vi "Event Handler.vi"(8 "error in":errorcluster, 11 "Listbox in":refnum<class "Multi Column Listbox.lvclass">) -> (0 "error out":errorcluster, 3 "Listbox out":refnum<class "Multi Column Listbox.lvclass">)   [LabVIEW 2013, in "Table Manager.lvlib" / "Multi Column Listbox.lvclass"]
doc: "Contains a loop and event structure to handle all common MCLB user interactions."
uses:
  Multi Column Listbox.lvclass
  Multi Column Listbox.lvclass/Multi Column Listbox.ctl
  Table Manager/Table Manager.lvclass/Table Manager.ctl
  <vilib>/Utility/miscctls.llb/LVPositionTypeDef.ctl
  <vilib>/Utility/miscctls.llb/LVRowAndColumnTypeDef.ctl
  Table Manager/Menu Select.ctl
  Table Manager/Read object refs.vi
  Table Manager/Read Menu Selection.vi
  Table Manager.lvlib
  Table Manager/Table Manager.lvclass
panel:
  out "Char":i16
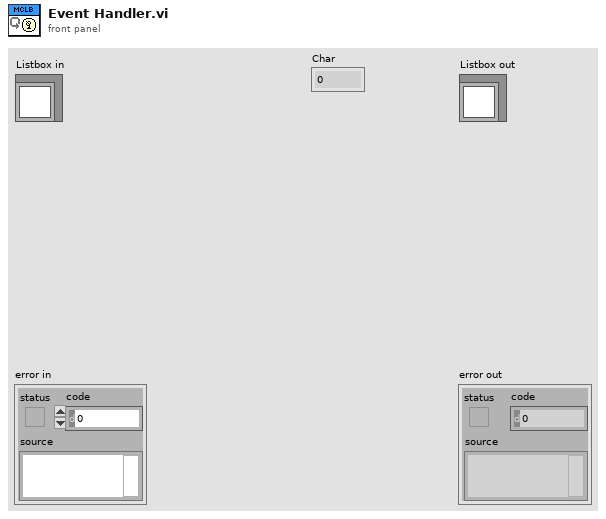
[diagram p1: front panel]
types:
  T1 = typedef "LVPositionTypeDef.ctl" = cluster{"Left":i32, "Top":i32}
  T2 = typedef "LVRowAndColumnTypeDef.ctl" = cluster{"Row":i32, "Column":i32}
  T3 = typedef "Table Manager.lvlib/Table Manager.lvclass/Menu Select.ctl" = cluster{"Line Name":string, "Selected Value":string, "Row":i32, "Column":i32, "Table Index":i32}
  T4 = typedef "Table Manager.lvlib/Table Manager.lvclass/object ref.ctl" = cluster{"engine":refnum<data-value>, "Node Ref":refnum<data-value>}
  T5 = typedef "NISE_CEF_Node.lvclass/RefreshUIEvent.ctl" = refnum<user-event>
  T6 = typedef "Table Manager.lvlib/Multi Column Listbox.lvclass/Int Reg Events.ctl" = refnum<event-registration>
  T7 = typedef "control module editor.lvclass/dialog output action.ctl" = enum16{"Tag Created", "Tag Selected", "Set Default", "disconnect"}
  T8 = typedef "Table Manager.lvlib/Table Manager.lvclass/Call Back Ref Type Def.ctl" = refnum<vi>
  T9 = typedef "LVPoint32TypeDef.ctl" = cluster{"Horizontal":i32, "Vertical":i32}
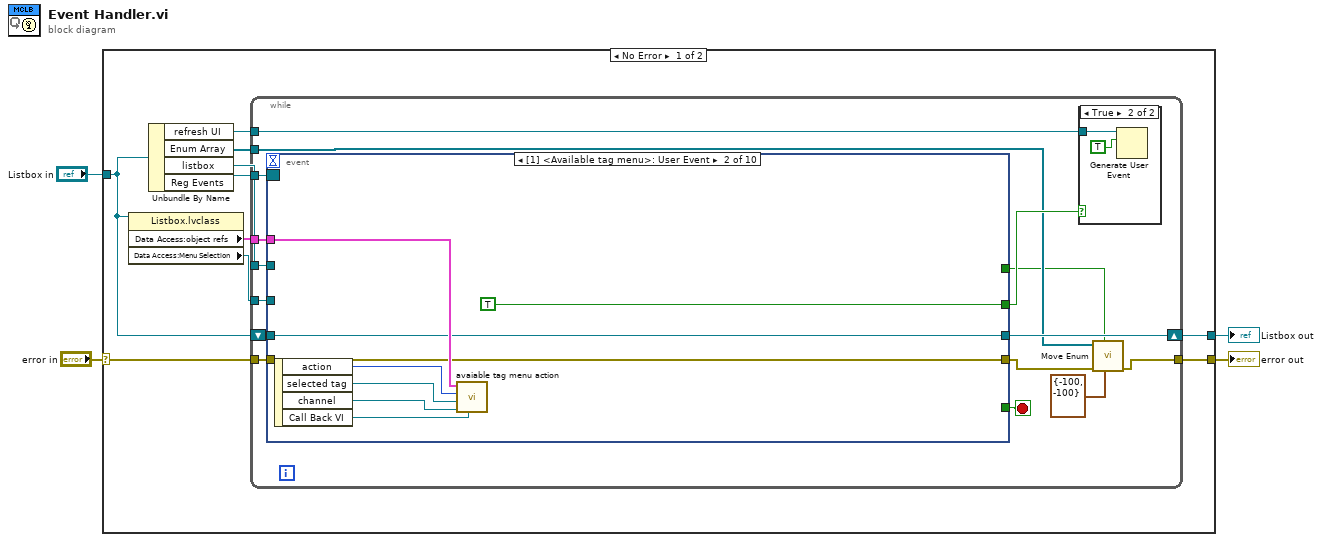
[diagram p0: block diagram]
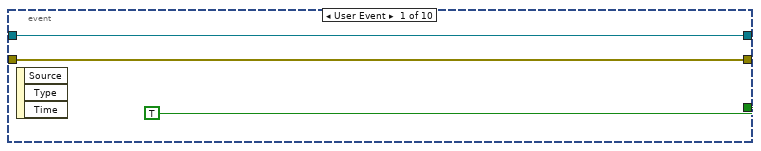
[diagram p3: hidden frame]
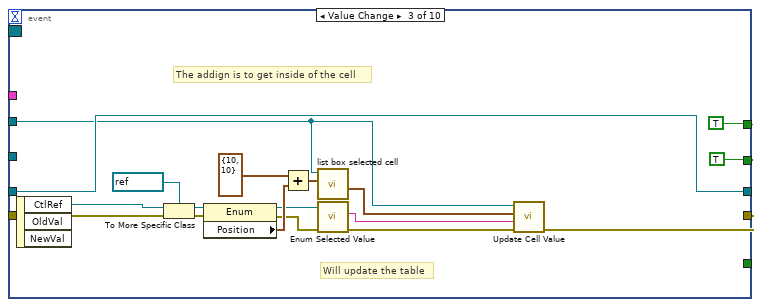
[diagram p4: hidden frame]
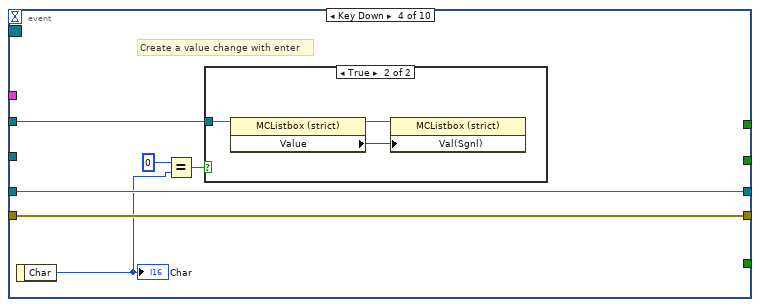
[diagram p5: hidden frame]
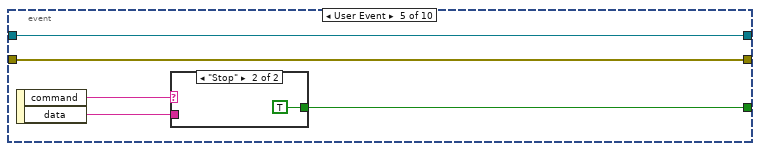
[diagram p7: hidden frame]
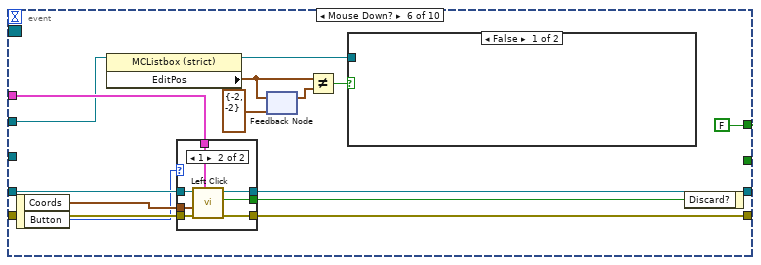
[diagram p9: hidden frame]
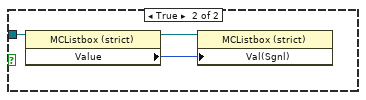
[diagram p10: hidden frame]
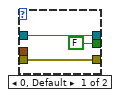
[diagram p11: hidden frame]
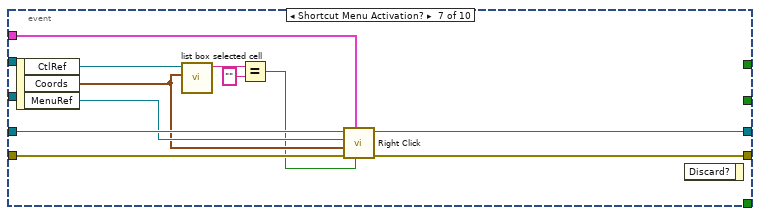
[diagram p12: hidden frame]
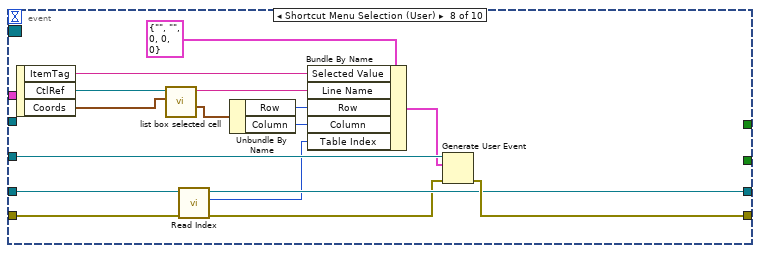
[diagram p13: hidden frame]
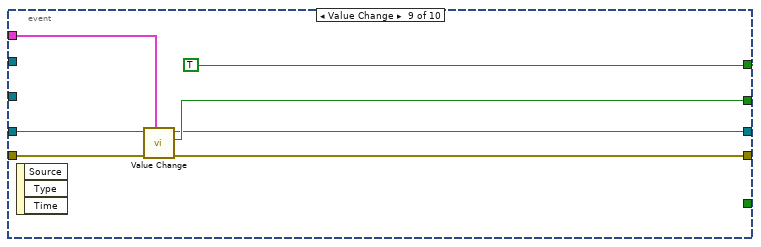
[diagram p14: hidden frame]
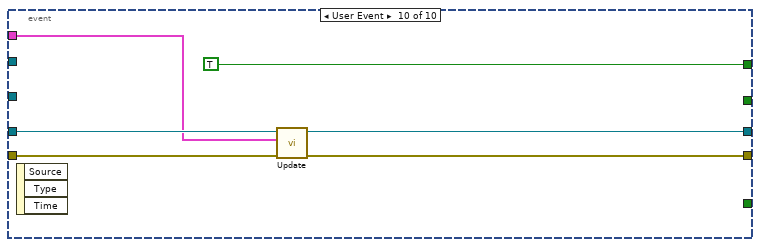
[diagram p15: hidden frame]
diagram:
  n1 = case shown="No Error" "error in" {
    selector: "error in" -> [w12 w145]
    tunnel: [w11 w145] -> w2
    tunnel: [w14 w144] -> w3
    tunnel: "Listbox in" -> [w7 w144]
    frame No Error {
      n2 = property class="Listbox.lvclass"(reference=w7) -> ("Data Access:object refs"=w6:T4, "Data Access:Menu Selection"=w5:refnum<user-event>)  [unwired: 1 in, 2 out]
      n3 = Unbundle By Name(w7) -> ("refresh UI"=w9:T5, "Enum Array"=w8:refnum<vi>[], "listbox"=w10:refnum<vi>, "Reg Events"=w13:T6)
      n4 = while {
        shift-right: [w25] -> w14
        shift-left: w7 -> [w26]
        tunnel: w13 -> [w28]
        tunnel: w6 -> [w27]
        tunnel: w12 -> [w24]
        tunnel: [w20] -> w11
        tunnel: w8 -> [w22]
        tunnel: w10 -> [w19]
        tunnel: w9 -> [w18]
        tunnel: w5 -> [w15]
        stop <- w29 stop-if-true
        n5 = event shown="[1] <Available tag menu>: User Event" {
          selector: w28 -> [_ _ _ _ _ _ _ _ _ _]
          dyn-events: _ -> [_ _ _ _ _ _ _ _ _ _]
          timeout: _ -> [_ _ _ _ _ _ _ _ _ _]
          tunnel: [TRUE _ _ _ w70 _ _ _ _ _] -> w29
          tunnel: w27 -> [_ w41 _ _ _ w89 w113 _ w133 w141]
          tunnel: w26 -> [w33 w40 w60 w66 w74 w84 w114 w119 w136 w143]
          tunnel: [w33 w40 w60 w66 w74 w90 w109 w118 w131 w142] -> w25
          tunnel: w24 -> [w32 w36 w49 w65 w73 w87 w112 w117 w135 w140]
          tunnel: [w32 w36 w47 w65 w73 w86 w111 w121 w134 w139] -> w21
          tunnel: [_ TRUE ("changed") TRUE ("changed") _ _ _ _ _ w132 _] -> w23
          tunnel: [_ _ TRUE _ _ FALSE _ _ TRUE TRUE] -> w16
          tunnel: w19 -> [_ _ w58 w61 _ w81 _ _ _ _]
          tunnel: w15 -> [_ _ _ _ _ _ _ w128 _ _]
          event User Event {
            n6 = event-data() -> ()  [unwired: 1 in, 3 out]
          }
          event User Event {
            n7 = event-data() -> ("action"=w42:T7, "selected tag"=w39:refnum<class "tag descriptor.lvclass">, "channel"=w38:refnum<class "TBM channel.lvclass">, "Call Back VI"=w35:T8)  [unwired: 1 in]
            n8 = call "avaiable tag menu action.vi"("Call Back VI"=w35, "channel"=w38, "selected tag"=w39, "action"=w42, "object ref"=w41) -> ()  [unwired: 5 in, 2 out]
          }
          event Value Change {
            # "Will update the table"
            # "The addign is to get inside of the cell"
            n9 = event-data() -> ("CtlRef"=w59:refnum<vi>)  [unwired: 1 in, 2 out]
            n10 = To More Specific Class(target class=refnum<vi> refnum ("Enum"), reference=w59, error in=w49) -> (specific class reference=w45:refnum<vi>, error out=w48:errorcluster)
            n11 = property class="Enum"(reference=w45, error in=w48) -> (reference out=w44:refnum<vi>, error out=w43:errorcluster, "Position"=w53:T1)
            n12 = Add(x=T1 {"Left"=10, "Top"=10} ("y"), y=w53) -> (x+y=w51:T1)
            n13 = call "list box selected cell.vi"("Coords"=w51, "MulticolumnListbox in"=w58) -> ("cell position"=w54:T2)  [unwired: 6 in, 3 out]
            n14 = call "Enum Selected Value.vi"("error in"=w43, "Enum"=w44) -> ("error out"=w46:errorcluster, "Value"=w50:string)  [unwired: 7 in, 1 out]
            n15 = call "Update Cell Value.vi"("error in"=w46, "Value"=w50, "cell position in"=w54, "MulticolumnListbox in"=w58) -> ("error out"=w47:errorcluster)  [unwired: 6 in, 1 out]
          }
          event Key Down {
            # "Create a value change with enter"
            n16 = event-data() -> ("Char"=w64:i16)  [unwired: 1 in]
            "Char" <- w64
            n17 = Equal?(x=i16 0, y=w64) -> (x = y?=w62:bool)
            n18 = case shown="True" w62 {
              tunnel: w61 -> [_ w69]
              frame False {
              }
              frame True {
                n19 = property class="MCListbox (strict)"(reference=w69) -> (reference out=w68:refnum<vi>, "Value"=w67:i32)  [unwired: 1 in, 1 out]
                n20 = property class="MCListbox (strict)"(reference=w68, "Val(Sgnl)"=w67) -> ()  [unwired: 1 in, 2 out]
              }
            }
          }
          event User Event {
            n21 = event-data() -> ("command"=w72:string, "data"=w71:string)  [unwired: 1 in]
            n22 = case shown="\"Stop\"" w72 {
              tunnel: [_ TRUE] -> w70
              tunnel: w71 -> [_ _]
              frame Default {
              }
              frame "Stop" {
              }
            }
          }
          event Mouse Down? {
            n23 = event-data() -> ("Coords"=w88:T9, "Button"=w82:u16)  [unwired: 1 in]
            n24 = property class="MCListbox (strict)"(reference=w81) -> (reference out=w76:refnum<vi>, "EditPos"=w80:T2)  [unwired: 1 in, 1 out]
            n25 = case shown="1" w82 {
              tunnel: [w96 w103] -> w90
              tunnel: w89 -> [_ w102]
              tunnel: w88 -> [_ w101]
              tunnel: w87 -> [w94 w100]
              tunnel: [w94 w99] -> w86
              tunnel: [FALSE ("Discard?") w98] -> w85
              tunnel: w84 -> [w96 w97]
              frame 0, Default {
              }
              frame 1 {
                n26 = call-dynamic "Left Click.vi"("object refs"=w102, "error in"=w100, "Coords"=w101, "Multi Column Listbox in"=w97) -> ("error out"=w99:errorcluster, "Discard?"=w98:bool, "Multi Column Listbox out"=w103:refnum<class "Multi Column Listbox.lvclass">)  [unwired: 5 in]
              }
            }
            n27 = feedback-in #1(w80) -> ()
            n28 = feedback #1(T2 {"Row"=-2, "Column"=-2} ("EditPos")) -> (w79:T2)
            n29 = Not Equal?(x=w80, y=w79) -> (x != y?=w77:bool)
            n30 = case shown="False" w77 {
              tunnel: w76 -> [_ w93]
              frame False {
              }
              frame True {
                n31 = property class="MCListbox (strict)"(reference=w93) -> (reference out=w92:refnum<vi>, "Value"=w91:i32)  [unwired: 1 in, 1 out]
                n32 = property class="MCListbox (strict)"(reference=w92, "Val(Sgnl)"=w91) -> ()  [unwired: 1 in, 2 out]
              }
            }
            n33 = event-data("Discard?"=w85) -> ()  [unwired: 1 in, 1 out]
          }
          event Shortcut Menu Activation? {
            n34 = event-data() -> ("CtlRef"=w108:refnum<vi>, "Coords"=w107:T9, "MenuRef"=w110:refnum<k9>)  [unwired: 1 in]
            n35 = call "list box selected cell.vi"("Coords"=w107, "MulticolumnListbox in"=w108) -> ("tag select name"=w106:string)  [unwired: 6 in, 3 out]
            n36 = Equal?(x=w106, y="") -> (x = y?=w104:bool)
            n37 = call-dynamic "Right Click.vi"("Empty Line?"=w104, "object refs"=w113, "error in (no error)"=w112, "Coords"=w107, "Event data"=w110, "Multi Column Listbox in"=w114) -> ("error out"=w111:errorcluster, "Multi Column Listbox out"=w109:refnum<class "Multi Column Listbox.lvclass">)  [unwired: 4 in]
            n38 = event-data() -> ()  [unwired: 2 in, 1 out]
          }
          event Shortcut Menu Selection (User) {
            n39 = event-data() -> ("ItemTag"=w120:string, "CtlRef"=w130:refnum<vi>, "Coords"=w129:T9)  [unwired: 1 in]
            n40 = call "list box selected cell.vi"("Coords"=w129, "MulticolumnListbox in"=w130) -> ("cell position"=w125:T2, "tag select name"=w126:string)  [unwired: 6 in, 2 out]
            n41 = call "Read Index.vi"("error in (no error)"=w117, "Table Manager in"=w119) -> ("error out"=w116:errorcluster, "Index"=w115:i32, "Table Manager out"=w118:refnum<class "Multi Column Listbox.lvclass">)  [unwired: 7 in]
            n42 = Unbundle By Name(w125) -> ("Row"=w124:i32, "Column"=w123:i32)
            n43 = Bundle By Name(cluster=T3 {"Line Name"="", "Selected Value"="", "Row"=0, "Column"=0, "Table Index"=0} ("event data"), "Selected Value"=w120, "Line Name"=w126, "Row"=w124, "Column"=w123, "Table Index"=w115) -> (w122:T3)
            n44 = Generate User Event(user event=w128, event data cluster=w122, error in=w116) -> (error out=w121:errorcluster)  [unwired: 1 in, 1 out]
          }
          event Value Change {
            n45 = event-data() -> ()  [unwired: 1 in, 3 out]
            n46 = call-dynamic "Value Change.vi"("objects"=w133, "error in"=w135, "Multi Column Listbox in"=w136) -> ("error out"=w134:errorcluster, "Update?"=w132:bool, "Multi Column Listbox out"=w131:refnum<class "Multi Column Listbox.lvclass">)  [unwired: 6 in]
          }
          event User Event {
            n47 = event-data() -> ()  [unwired: 1 in, 3 out]
            n48 = call-dynamic "Update.vi"("error in"=w140, "object ref in"=w141, "Multi Column Listbox in"=w143) -> ("error out"=w139:errorcluster, "Multi Column Listbox out"=w142:refnum<class "Multi Column Listbox.lvclass">)  [unwired: 6 in, 1 out]
          }
        }
        n49 = case shown="True" w23 {
          tunnel: w18 -> [_ w30]
          frame False {
          }
          frame True {
            n50 = Generate User Event(user event=w30, event data cluster=TRUE ("event data")) -> ()  [unwired: 2 in, 2 out]
          }
        }
        n51 = call "Move Enum.vi"("position"=T1 {"Left"=-100, "Top"=-100}, "move?"=w16, "error in"=w21, "Enum Array"=w22) -> ("error out"=w20:errorcluster)  [unwired: 7 in]
      }
    }
    frame Error {
    }
  }
  "error out" <- w2
  "Listbox out" <- w3
